vi "Get FilterDelay.vi"(8 "error in (no error)":errorcluster, 10 "SampClk.Rate":dbl, 11 "DAQ Type":T1) -> (0 "error out":errorcluster, 1 "Total Delay":dbl, 2 "DAC Delay (samples)":dbl, 3 "ADC Delay (samples)":dbl)   [LabVIEW 2019, in "DAQmx.lvclass"]
uses:
  DAQmx.lvclass
  typedefs/DAQmx.Config.Device Type--enum.ctl
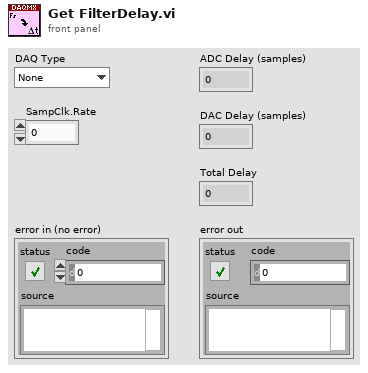
[diagram p1: front panel]
types:
  T1 = typedef "DAQmx.lvclass/DAQmx.Config.Device Type--enum.ctl" = enum16{"None", "USB-4431", "PXI-446x"}
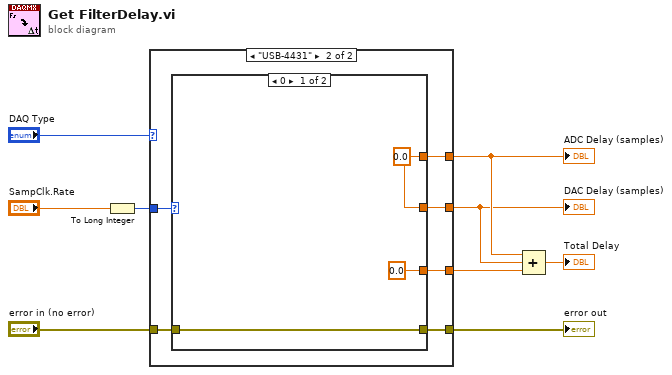
[diagram p0: block diagram]
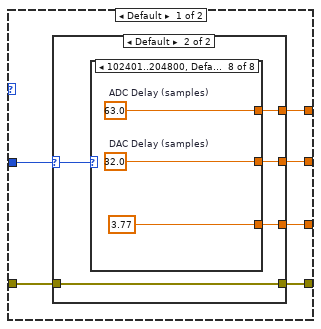
[diagram p2: hidden frame]
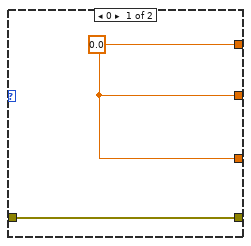
[diagram p3: hidden frame]
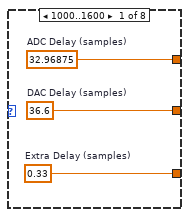
[diagram p4: hidden frame]
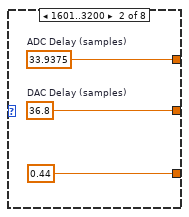
[diagram p5: hidden frame]
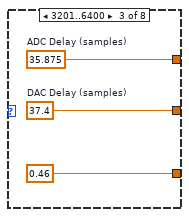
[diagram p6: hidden frame]
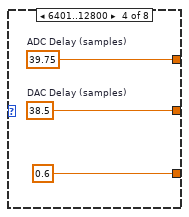
[diagram p7: hidden frame]
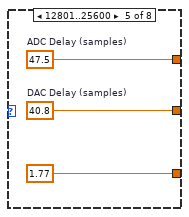
[diagram p8: hidden frame]
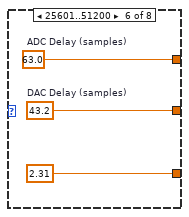
[diagram p9: hidden frame]
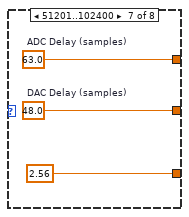
[diagram p10: hidden frame]
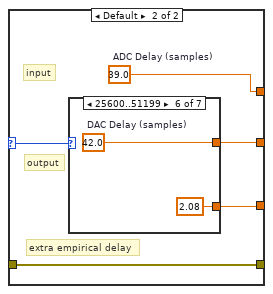
[diagram p11: hidden frame]
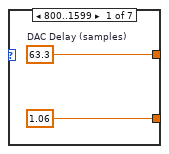
[diagram p12: hidden frame]
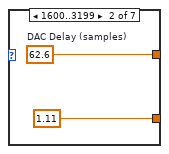
[diagram p13: hidden frame]
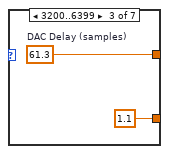
[diagram p14: hidden frame]
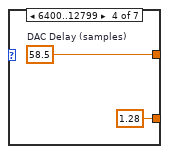
[diagram p15: hidden frame]
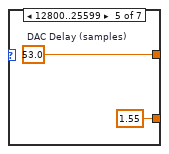
[diagram p16: hidden frame]
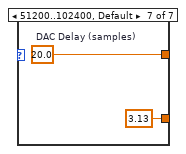
[diagram p17: hidden frame]
diagram:
  n1 = To Long Integer(number="SampClk.Rate") -> (32bit integer=w7:i32)
  n2 = case shown="\"USB-4431\"" "DAQ Type" {
    tunnel: w7 -> [w10 w48]
    tunnel: [w15 w52] -> w8
    tunnel: [w14 w51] -> w9
    tunnel: "error in (no error)" -> [w13 w50]
    tunnel: [w12 w49] -> w1
    tunnel: [w11 w47] -> w5
    frame Default {
      n3 = case shown="Default" w10 {
        selector: w10 -> [_ w18]
        tunnel: [w16 w22] -> w15
        tunnel: [w16 w21] -> w14
        tunnel: w13 -> [w17 w20]
        tunnel: [w17 w20] -> w12
        tunnel: [w16 w19] -> w11
        frame 0 {
          w16 = 0.0 ("ADC Delay (samples)")
        }
        frame Default {
          n4 = case shown="102401..204800, Default" w18 {
            tunnel: [w25 w28 w31 w34 w37 w40 w43 w46] -> w21
            tunnel: [w24 w27 w30 w33 w36 w39 w42 w45] -> w22
            tunnel: [w23 0.44 ("Extra Delay (samples)") 0.46 ("Extra Delay (samples)") 0.6 ("Extra Delay (samples)") 1.77 ("Extra Delay (samples)") 2.31 ("Extra Delay (samples)") 2.56 ("Extra Delay (samples)") 3.77 ("Extra Delay (samples)")] -> w19
            frame 1000..1600 {
              w23 = 0.33  # Extra Delay (samples)
              w24 = 36.6  # DAC Delay (samples)
              w25 = 32.96875  # ADC Delay (samples)
            }
            frame 1601..3200 {
              w27 = 36.8  # DAC Delay (samples)
              w28 = 33.9375  # ADC Delay (samples)
            }
            frame 3201..6400 {
              w30 = 37.4  # DAC Delay (samples)
              w31 = 35.875  # ADC Delay (samples)
            }
            frame 6401..12800 {
              w33 = 38.5  # DAC Delay (samples)
              w34 = 39.75  # ADC Delay (samples)
            }
            frame 12801..25600 {
              w36 = 40.8  # DAC Delay (samples)
              w37 = 47.5  # ADC Delay (samples)
            }
            frame 25601..51200 {
              w40 = 63.0  # ADC Delay (samples)
              w39 = 43.2  # DAC Delay (samples)
            }
            frame 51201..102400 {
              w43 = 63.0  # ADC Delay (samples)
              w42 = 48.0  # DAC Delay (samples)
            }
            frame 102401..204800, Default {
              w46 = 63.0  # ADC Delay (samples)
              w45 = 32.0  # DAC Delay (samples)
            }
          }
        }
      }
    }
    frame "USB-4431" {
      n5 = case shown="0" w48 {
        selector: w48 -> [_ w58]
        tunnel: [w55 w60] -> w52
        tunnel: [w55 w57] -> w51
        tunnel: w50 -> [w54 w59]
        tunnel: [w54 w59] -> w49
        tunnel: [0.0 ("Extra Delay (samples)") w56] -> w47
        frame 0 {
          w55 = 0.0 ("ADC Delay (samples)")
        }
        frame Default {
          w57 = 39.0  # ADC Delay (samples)
          # "extra empirical delay"
          # "input"
          # "output"
          n6 = case shown="25600..51199" w58 {
            tunnel: [w62 w64 w66 w68 w70 w72 w74] -> w60
            tunnel: [1.06 ("Extra Delay (samples)") 1.11 ("Extra Delay (samples)") 1.1 ("Extra Delay (samples)") 1.28 ("Extra Delay (samples)") 1.55 ("Extra Delay (samples)") 2.08 ("Extra Delay (samples)") 3.13 ("Extra Delay (samples)")] -> w56
            frame 800..1599 {
              w62 = 63.3  # DAC Delay (samples)
            }
            frame 1600..3199 {
              w64 = 62.6  # DAC Delay (samples)
            }
            frame 3200..6399 {
              w66 = 61.3  # DAC Delay (samples)
            }
            frame 6400..12799 {
              w68 = 58.5  # DAC Delay (samples)
            }
            frame 12800..25599 {
              w70 = 53.0  # DAC Delay (samples)
            }
            frame 25600..51199 {
              w72 = 42.0  # DAC Delay (samples)
            }
            frame 51200..102400, Default {
              w74 = 20.0  # DAC Delay (samples)
            }
          }
        }
      }
    }
  }
  "ADC Delay (samples)" <- w9
  "DAC Delay (samples)" <- w8
  "error out" <- w1
  n7 = Compound Arithmetic op=ADD(w9, w8, w5) -> (→"Total Delay":dbl)
